vi "csm_agent_bridge_add_state.vi"(8 "New State Name":string, 11 "Target VI Path":string) -> (0 "error out":errorcluster)   [LabVIEW 2025]
uses:
  <userlib>/_NEVSTOP/Communicable State Machine(CSM)/_csmHelper/API/Open Block Diagram.vi
  <userlib>/_NEVSTOP/Communicable State Machine(CSM)/_csmHelper/CSM-Helper.lvclass
  <userlib>/_NEVSTOP/Communicable State Machine(CSM)/_csmHelper/API/Connect Paired Tunnels.vi
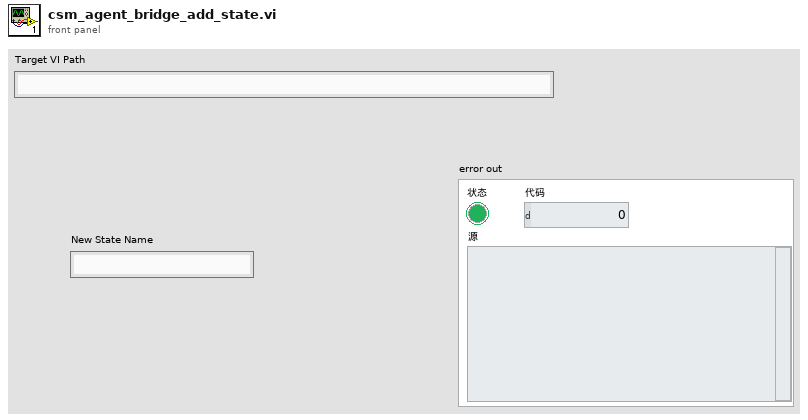
[diagram p1: front panel]
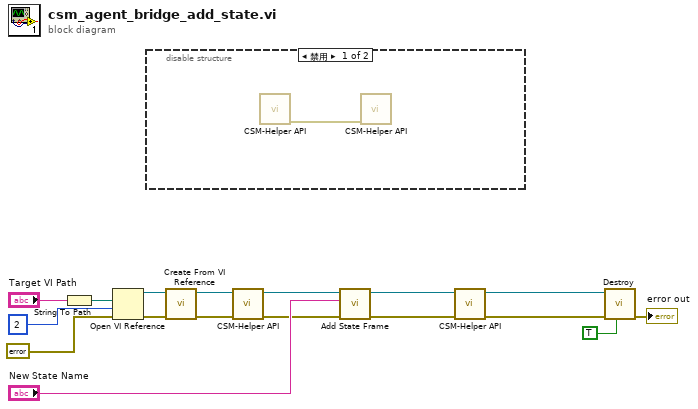
[diagram p0: block diagram]
diagram:
  n1 = String To Path(string="Target VI Path") -> (path=w5:path)
  n2 = Open VI Reference(vi path=w5, options=2, error in (no error)=errorcluster {"status"=FALSE, "code"=0, "source"=""} ("错误输入（无错误）")) -> (vi reference=w14:refnum<vi>, error out=w12:errorcluster)  [unwired: 3 in]
  n3 = disable-structure shown="禁用" {
    frame Disabled {
      n4 = call-poly <userlib>:"CSM-Helper API.vi"() -> ("error out"=w18:errorcluster)  [unwired: 9 in, 2 out]
      n5 = call-poly <userlib>:"CSM-Helper API.vi"("error in (no error)"=w18) -> ()  [unwired: 9 in, 2 out]
    }
    frame Enabled {
    }
  }
  n6 = call <userlib>:"Create From VI Reference.vi"("error in (no error)"=w12, "VI"=w14) -> ("error out"=w9:errorcluster, "CSM-Helper.lvclass"=w10:refnum<class "CSM-Helper.lvclass">)  [unwired: 8 in]
  n7 = call-poly <userlib>:"CSM-Helper API.vi"("error in (no error)"=w9, "CSM-Helper in"=w10) -> ("error out"=w7:errorcluster, "CSM-Helper out"=w8:refnum<class "CSM-Helper.lvclass">)  [unwired: 8 in]
  n8 = call <userlib>:"Add State Frame.vi"("error in (no error)"=w7, "element"="New State Name", "CSM-Helper in"=w8) -> ("error out"=w3:errorcluster, "CSM-Helper out"=w4:refnum<class "CSM-Helper.lvclass">)  [unwired: 6 in, 1 out]
  n9 = call-poly <userlib>:"CSM-Helper API.vi"("error in (no error)"=w3, "CSM-Helper in"=w4) -> ("error out"=w1:errorcluster, "CSM-Helper out"=w2:refnum<class "CSM-Helper.lvclass">)  [unwired: 8 in]
  n10 = call <userlib>:"Destroy.vi"("Save Instruments?(F)"=TRUE, "error in (no error)"=w1, "CSM-Helper in"=w2) -> ("error out"=→"error out":errorcluster)  [unwired: 7 in, 1 out]
